vi "VHistory - Preset CDB Scalar History.vi"(5 "writer IDs":u32[](array[numeric]), 6 "append (F)":bool, 7 "VC Handle":T1=-1, 8 "error in":errorcluster, 9 "history":cdb[](array[numeric]), 10 "time stamps":dbl[](array[numeric]) format="%<%H:%M:%S%2u\n%d/%m/%Y>T", 11 "name_spec":string) -> (0 "error out":errorcluster, 3 "dup name_spec":string)   [LabVIEW 2021]
doc: "This VI presets the history of a variable of the <b>CDB Number</b> data type. It can either set new history data or append new data to the existing history. This VI sorts timestamps, history values, and writer IDs in ascending chronological order before it presets them to the history; however, the VI does not sort the history after appending the new data. Refer to the VI help for more details.\n\n<b>VC Handle</b> and <b>name_spec</b> controls specify the desired variable. The variable must exist and have a history attached; otherwise, the VI returns an error. Use <b>VHistory - History Controller.vi</b> to attach a history to a variable.\n\n<b>VC Handle</b> specifies the handle of the variable context. To operate on a global variable, pass -1 to this input. This input is ignored if the <b>name_spec</b> control refers to a variable by an alias.\n\n<b>name_spec</b> is the name specifier of the desired variable. Usually, it is merely a variable name; however, its generic format is '[name][=alias]', where either 'name' or '=alias' can be omitted but not both.\n\n<b>history</b> control specifies the history values to be preset.\n\n<b>time stamps</b> control specifies the timestamps, in the standard LabVIEW date/time format, of the respective elements in <b>history</b>.\n\n<b>writer IDs</b> control specifies the IDs of the writers for the respective elements in <b>history</b>. If the history does not store writer IDs, this input is ignored. If the size of this array is less than the size of <b>history</b> and <b>time stamps</b>, its first element is bound to all new history values.\n\n<b>append</b> control specifies whether to append new history data. If FALSE (default), the VI discards old history data and presets the new data to the history. If TRUE, the VI appends the new data to the end of the existing history. Note that appending data can break the chronological order of the history if the new timestamps are older than timestamps in the history.\n\n::: CalcExpress Toolkit :::\nCopyright (c) 2000-2026 Konstantin Shifershteyn. All rights reserved."
uses:
  cetypes.llb/VarMan Variable Context Handle.ctl
  cetypes.llb/CalcExpress Data Type.ctl
  cersrc/celveng32.dll
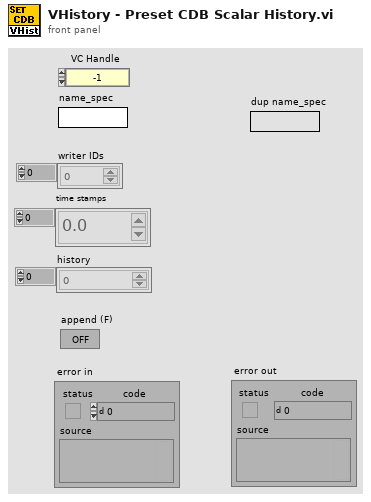
[diagram p1: front panel]
types:
  T1 = typedef "VarMan Variable Context Handle.ctl" = i32
  T2 = typedef "CalcExpress Data Type.ctl" = enum32{"String", "DBL Number", "identifier", "1D Array of DBL", "2D Array of DBL", "CDB Number", "1D Array of CDB", "2D Array of CDB", "1D Array of String", "2D Array of String", "Unknown data type"}
  T3 = enum16{"big-endian, network order", "native, host order", "little-endian"}
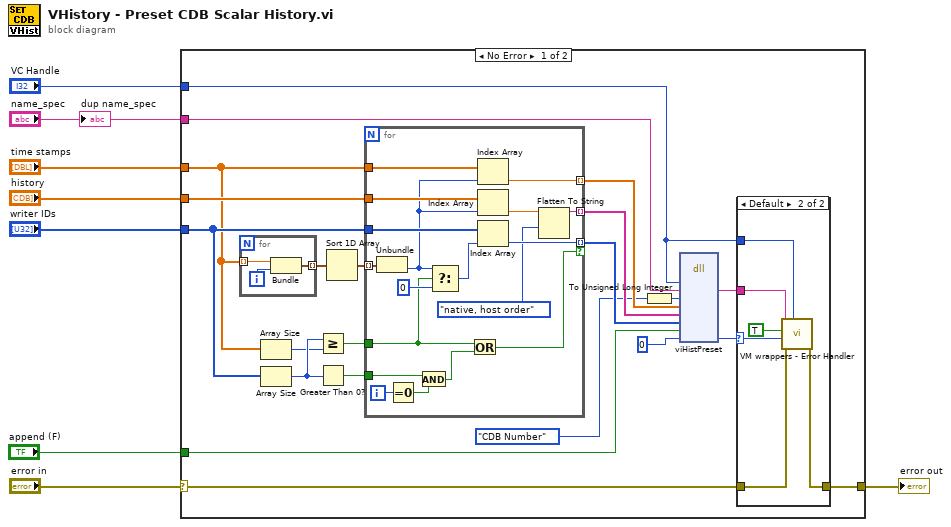
[diagram p0: block diagram]
diagram:
  n1 = case shown="No Error" "error in" {
    selector: "error in" -> [w13 w59]
    tunnel: "name_spec" -> [w29 _]
    tunnel: "VC Handle" -> [w12 _]
    tunnel: [w28 w59] -> w1
    tunnel: "time stamps" -> [w17 _]
    tunnel: "history" -> [w24 _]
    tunnel: "append (F)" -> [w20 _]
    tunnel: "writer IDs" -> [w18 _]
    frame No Error {
      n2 = for {
        tunnel: w17 -> [w50] mode=indexing
        tunnel: [w49] -> w25 mode=indexing
        i -> [w51]
        n3 = Bundle("timestamp"=w50, w51) -> (w49:cluster{"timestamp":dbl, i32})  [unwired: 1 in]
      }
      n4 = Array Size(array=w17) -> (size(s)=w9:i32)
      n5 = Array Size(array=w18) -> (size(s)=w10:i32)
      n6 = Greater Or Equal?(x=w10, y=w9) -> (x >= y?=w16:bool)
      n7 = Greater Than 0?(x=w10) -> (x > 0?=w15:bool)
      n8 = Sort 1D Array(array=w25) -> (sorted array=w23:cluster{"timestamp":dbl, i32}[])
      n9 = for {
        tunnel: w17 -> [w48]
        tunnel: w24 -> [w47]
        tunnel: w23 -> [w46] mode=indexing
        tunnel: [w45] -> w22 mode=indexing
        tunnel: [w36] -> w21 mode=indexing
        tunnel: w18 -> [w44]
        tunnel: [w43] -> w19 mode=indexing if=w42
        tunnel: w16 -> [w32]
        tunnel: w15 -> [w40]
        i -> [w41]
        n10 = Unbundle(w46) -> (w33:i32)  [unwired: 1 out]
        n11 = Equal To 0?(x=w41) -> (x = 0?=w39:bool)
        n12 = And(x=w40, y=w39) -> (x .and. y?=w38:bool)
        n13 = Select(t=w33, s=w32, f=0 ("t")) -> (s? t:f=w31:i32)
        n14 = Or(x=w32, y=w38) -> (x .or. y?=w42:bool)
        n15 = Index Array(array=w48, index=w33) -> (element=w45:dbl)
        n16 = Index Array(array=w47, index=w33) -> (element=w37:cdb)
        n17 = Index Array(array=w44, index=w31) -> (element=w43:u32)
        n18 = Flatten To String(anything=w37, byte order (0:big-endian, network order)=T3."native, host order") -> (data string=w36:string)  [unwired: 2 in, 2 out]
      }
      n19 = To Unsigned Long Integer(number=CalcExpress_Data_Type."CDB Number" ("data type")) -> (unsigned 32bit integer=w30:u32)
      n20 = dll-call lib="C:/LV Projects/CalcExpress 40 LV2021/vi.lib/addons/CalcExpress/cersrc/celveng*.dll" fn="viHistPreset"("vch"=w12, "name"=w29, "type"=w30, "time"=w22, "data"=w21, "writerIDs"=w19, "append"=w20, "errc"=u16 0) -> ("name"=w26:string, "errc"=w14:u16)  [unwired: 10 in, 2 out]
      n21 = case shown="Default" w14 {
        selector: w14 -> [_ w54]
        tunnel: [w52 w58] -> w28
        tunnel: w26 -> [_ w56]
        tunnel: w12 -> [_ w55]
        tunnel: w13 -> [w52 w53]
        frame 0 {
        }
        frame Default {
          n22 = call "VM wrappers - Error Handler.vi"("VC Handle"=w55, "error before"=w53, "VarMan error"=w54, "show name spec (F)"=TRUE, "name spec"=w56) -> ("error out"=w58:errorcluster)  [unwired: 5 in, 1 out]
        }
      }
    }
    frame Error {
    }
  }
  "error out" <- w1
  "dup name_spec" <- "name_spec"
